vi "Shutdown.vi"(8 "error in (no error)":errorcluster, 11 "JKI_Python_Server in":refnum<class "Server.lvclass">) -> (0 "error out":errorcluster)   [LabVIEW 2020, in "jki_python_bridge.lvlib" / "Server.lvclass"]
uses:
  Server.lvclass
  Server.lvclass/Server.ctl
  PyObject/PyObject.lvclass
  <vilib>/addons/_JKI.lib/_JKI_lib_TCP_Server.llb/JKI TCP Server.lvclass
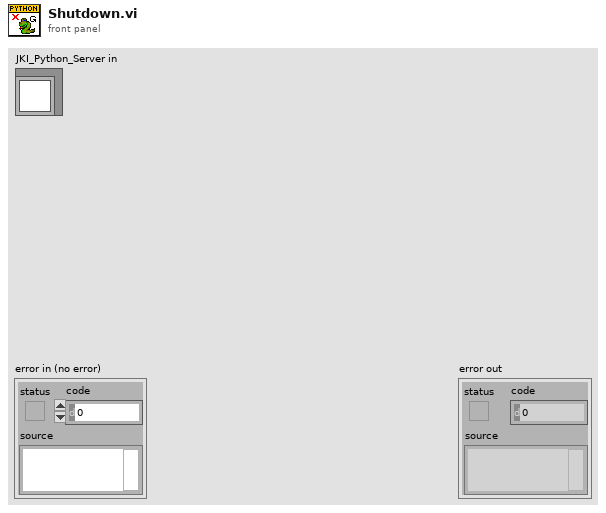
[diagram p1: front panel]
types:
  T1 = typedef "jki_python_bridge.lvlib/Server.lvclass/Class Private Data - Cluster.ctl" = cluster{"TCP Server Refnum":refnum<class "JKI TCP Server.lvclass">, "TCP port (50007)":u16, "max connections (0: no limit)":u32, "net address (0: Listen on All Adaptors)":u32, "Nodes":T2[], "Public Events":T3}
  T2 = typedef "jki_python_bridge.lvlib/Server.lvclass/Python Node.ctl" = cluster{"Name":string, "Python Method Call":refnum<user-event>, "Call Handle":refnum<class "PyObject.lvclass">}
  T3 = typedef "jki_python_bridge.lvlib/Server.lvclass/Public Events - Cluster.ctl" = cluster{"Stop Nodes":refnum<user-event>}
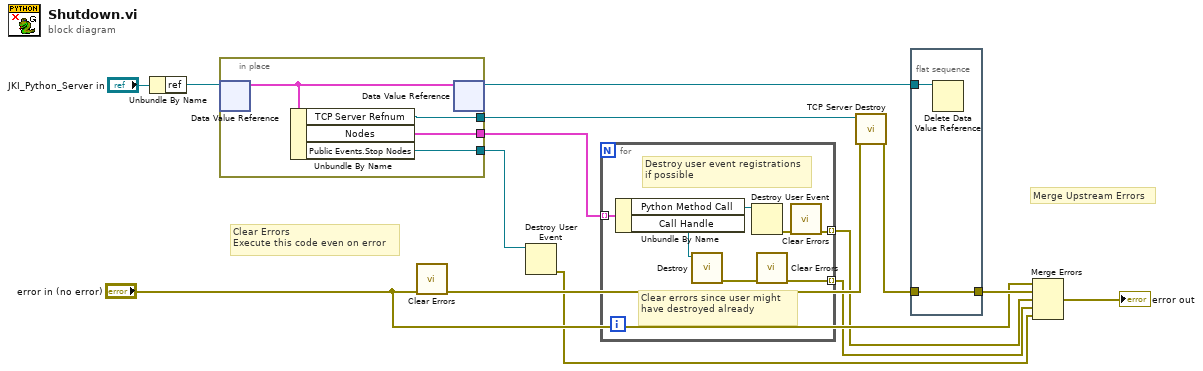
[diagram p0: block diagram]
diagram:
  # "Merge Upstream Errors"
  # "Clear Errors\nExecute this code even on error"
  n1 = Unbundle By Name("JKI_Python_Server in") -> ("ref"=w7:refnum<data-value>)
  n2 = in-place {
    in-place-border: [w18] -> w13
    in-place-border: [w16] -> w5
    in-place-border: [w15] -> w3
    n3 = in-place-dvr #1(w7) -> (w17:T1)  [unwired: 1 out]
    n4 = Unbundle By Name(w17) -> ("TCP Server Refnum"=w18:refnum<class "JKI TCP Server.lvclass">, "Nodes"=w16:T2[], "Public Events.Stop Nodes"=w15:refnum<user-event>)
    n5 = in-place-dvr #1(w17) -> (w6:refnum<data-value>)  [unwired: 1 out]
  }
  n6 = call <vilib>:"Clear Errors.vi"("error in (no error)"="error in (no error)") -> ("error out"=w11:errorcluster)  [unwired: 5 in, 1 out]
  n7 = Destroy User Event(user event=w3) -> (error out=w2:errorcluster)  [unwired: 1 in]
  n8 = for {
    tunnel: w5 -> [w25] mode=indexing
    tunnel: [w19] -> w4 mode=indexing
    tunnel: [w23] -> w1 mode=indexing
    # "Clear errors since user might have destroyed already"
    # "Destroy user event registrations\nif possible"
    n9 = Unbundle By Name(w25) -> ("Python Method Call"=w24:refnum<user-event>, "Call Handle"=w22:refnum<class "PyObject.lvclass">)
    n10 = call "Destroy.vi"("CallHandler in"=w22) -> ("error out"=w21:errorcluster)  [unwired: 10 in]
    n11 = Destroy User Event(user event=w24) -> (error out=w20:errorcluster)  [unwired: 1 in]
    n12 = call <vilib>:"Clear Errors.vi"("error in (no error)"=w21) -> ("error out"=w23:errorcluster)  [unwired: 5 in, 1 out]
    n13 = call <vilib>:"Clear Errors.vi"("error in (no error)"=w20) -> ("error out"=w19:errorcluster)  [unwired: 5 in, 1 out]
  }
  n14 = call <vilib>:"TCP Server Destroy.vi"("error in (no error)"=w11, "TCP Server"=w13) -> ("error out"=w12:errorcluster)  [unwired: 9 in]
  n15 = flat-sequence {
    tunnel: [w27] -> w14
    tunnel: w12 -> [w27]
    tunnel: w6 -> [w26]
    frame #0 {
      n16 = Delete Data Value Reference(data value reference=w26) -> ()  [unwired: 1 in, 2 out]
    }
  }
  n17 = Merge Errors("error in (no error)", w14, w4, w1, w2) -> (→"error out":errorcluster)
